vi "AR Table save for TDMS.vi"(8 "error in":errorcluster caption="エラー入力", 9 "AR Table Data":string[](array[string]), 10 "AR Table Tag":string[](array[string]), 11 "TDMSファイル in":refnum<k34>) -> (0 "error out":errorcluster, 3 "TDMSファイル out":refnum<k34>)   [LabVIEW 2018]
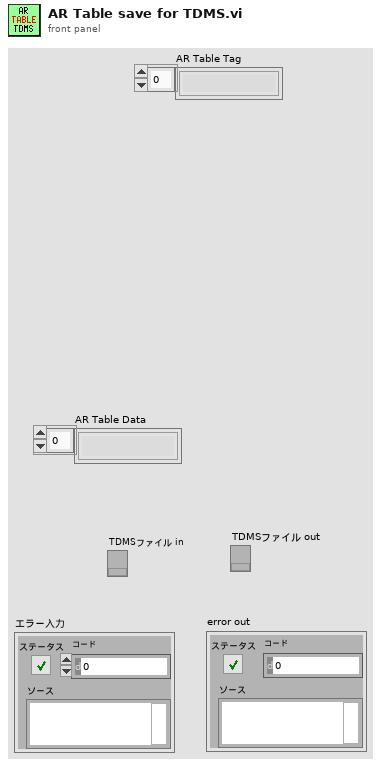
[diagram p1: front panel]
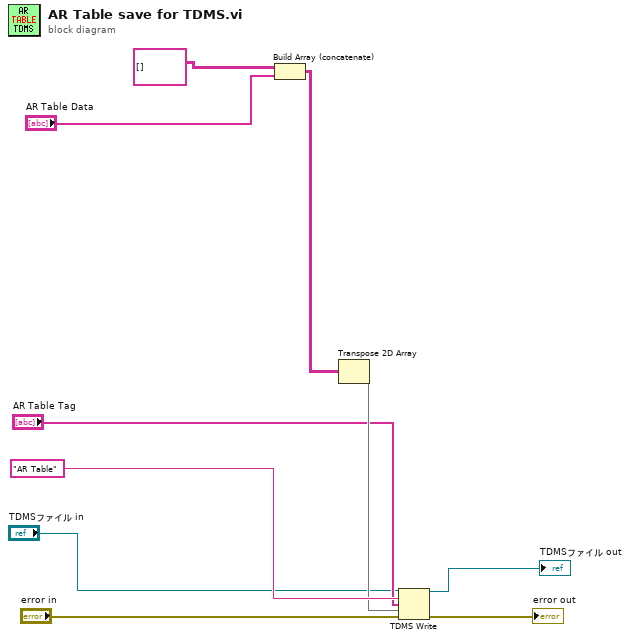
[diagram p0: block diagram]
diagram:
  n1 = Build Array (concatenate)(string[][] [] ("Table"), "AR Table Data") -> (w5:string[][])
  n2 = Transpose 2D Array(2D array=w5) -> (transposed array=w7:string[][])
  n3 = TDMS Write(0:"TDMSファイル in", 5:"AR Table" ("Group name"), 7:"AR Table Tag", 9:w7, 11:"error in") -> (4:→"TDMSファイル out":refnum<k34>, 15:→"error out":errorcluster)  [unwired: 1 in, 2 out]
